vi "Remove_File.vi"(8 "error in":errorcluster, 10 "file name":string, 11 "folder ready":path) -> (0 "error out":errorcluster)   [LabVIEW 2025]
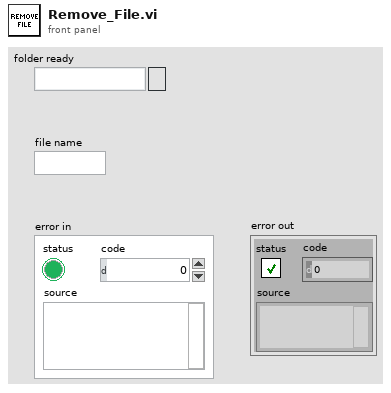
[diagram p1: front panel]
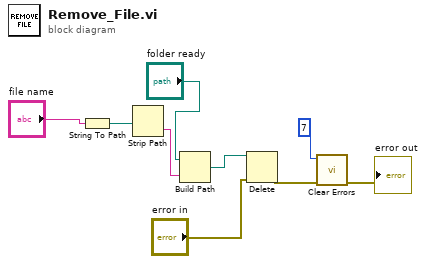
[diagram p0: block diagram]
diagram:
  n1 = String To Path(string="file name") -> (path=w6:path)
  n2 = Strip Path(path=w6) -> (name=w7:string)  [unwired: 1 out]
  n3 = Build Path(base path="folder ready", name or relative path=w7) -> (appended path=w9:path)
  n4 = Delete(path (use dialog)=w9, error in="error in") -> (error out=w3:errorcluster)  [unwired: 3 in, 2 out]
  n5 = call <vilib>:"Clear Errors.vi"("error in (no error)"=w3, "specific error code to clear (0: all)"=7) -> ("error out"=→"error out":errorcluster)  [unwired: 4 in, 1 out]
